vi "Get Local Chassis Slots Configuration.vi"(8 "error in (no error)":errorcluster, 11 "Item Ref in":T2 format="%.0x") -> (0 "error out":errorcluster, 2 "Slots Configuration":T1[](array[typedef]), 3 "Item Ref out":T2 format="%.0x")   [LabVIEW 2027, in "SEECD System Explorer.lvlib"]
doc: "This VI lists the module(s) configured in Local Chassis. GUIDs are used to create the list. The output is a list of Slot Number."
uses:
  SEECD System Explorer.lvlib
  <vilib>/NI VeriStand/Custom Device API/Custom Device Item Ref.ctl
  Type Defs/Slot Programming Mode.ctl
  Shared/Globals/Scan Engine GUIDs.vi
  <vilib>/NI VeriStand/Custom Device Tools/Custom Device Utility Library/NI VeriStand - Search for Item by GUID.vi
  Shared/Globals/Property Strings.vi
  <vilib>/NI VeriStand/Custom Device Tools/Custom Device Utility Library/Custom Device Utility Library.lvlib
  Shared/SEECD Shared.lvlib
  <vilib>/NI VeriStand/Custom Device API/Custom Device API.lvlib
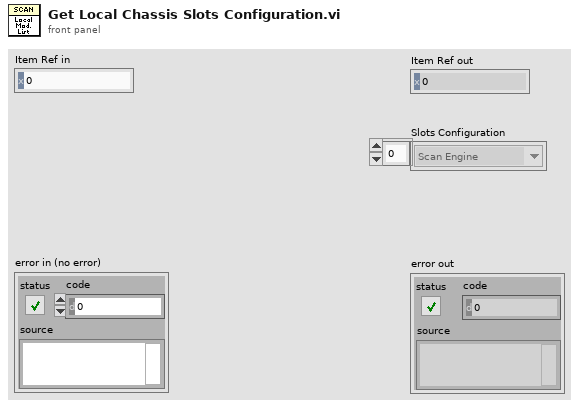
[diagram p1: front panel]
types:
  T1 = typedef "SEECD System Explorer.lvlib/Slot Programming Mode.ctl" = enum16{"Don't Modify", "Scan Engine", "LabVIEW FPGA", "NI-DAQmx"}
  T2 = typedef "Custom Device API.lvlib/Custom Device Item Ref.ctl" = u64
  T3 = typedef "Custom Device API.lvlib/Custom Device Item Info.ctl" = cluster{"Name":string, "Is Channel":bool, "GUID":string, "Is Waveform":bool}
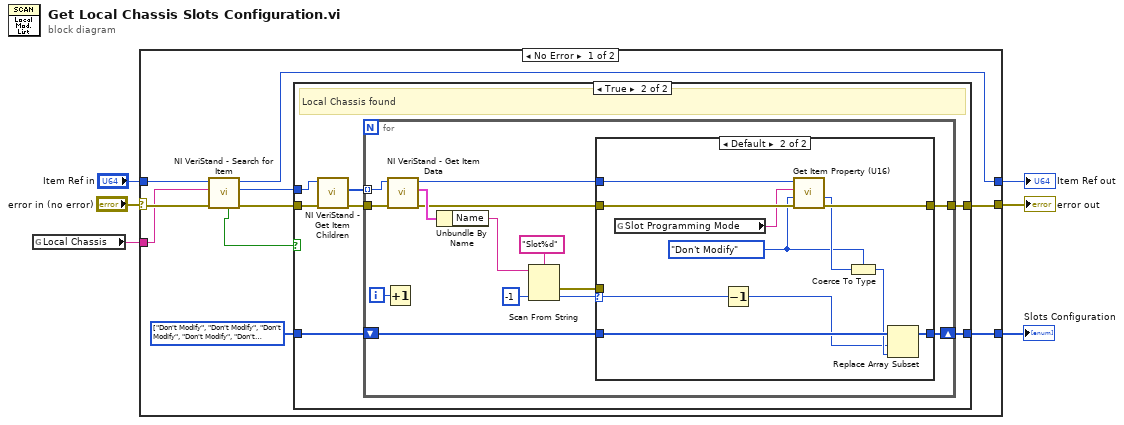
[diagram p0: block diagram]
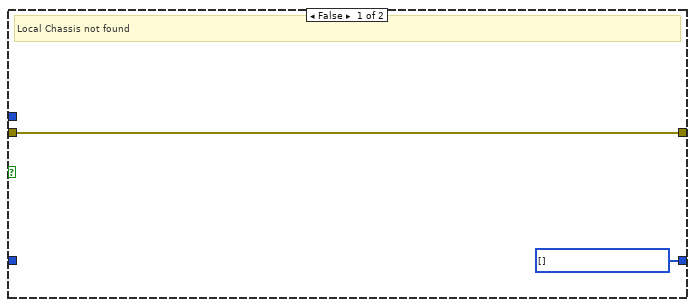
[diagram p2: hidden frame]
diagram:
  n1 = global read "Scan Engine GUIDs.vi" "Local Chassis"() -> (w3:string)
  n2 = case shown="No Error" "error in (no error)" {
    selector: "error in (no error)" -> [w16 w54]
    tunnel: [w9 w54] -> w5
    tunnel: "Item Ref in" -> [w15 w53]
    tunnel: w3 -> [w14 _]
    tunnel: [w10 w53] -> w2
    tunnel: [w8 _] -> w1
    frame No Error {
      w7 = T1[] [enum."Don't Modify", enum."Don't Modify", enum."Don't Modify", enum."Don't Modify", enum."Don't Modify", enum."Don't Modify", enum."Don't Modify", enum."Don't Modify"] items=["Don't Modify", "Scan Engine", "LabVIEW FPGA", "NI-DAQmx"] ("Slots Configuration")
      n3 = call-poly <vilib>:"NI VeriStand - Search for Item.vi"("error in"=w16, "Item GUID"=w14, "Section Ref in"=w15) -> ("error out"=w12:errorcluster, "Item Ref"=w11:T2, "Section Ref out"=w10:T2, "Found"=w13:bool)  [unwired: 5 in]
      n4 = case shown="True" w13 {
        tunnel: w12 -> [w18 w24]
        tunnel: w11 -> [_ w23]
        tunnel: [w18 w25] -> w9
        tunnel: [w17 w19] -> w8
        tunnel: w7 -> [_ w20]
        frame False {
          w17 = T1[] [] items=["Don't Modify", "Scan Engine", "LabVIEW FPGA", "NI-DAQmx"] ("Slots Configuration")
          # "Local Chassis not found"
        }
        frame True {
          # "Local Chassis found"
          n5 = call <vilib>:"NI VeriStand - Get Item Children.vi"("error in (no error)"=w24, "Item Ref in"=w23) -> ("error out"=w21:errorcluster, "Child Refs"=w22:T2[])  [unwired: 6 in, 2 out]
          n6 = for {
            tunnel: [w39] -> w25
            tunnel: w22 -> [w37] mode=indexing
            tunnel: w21 -> [w38]
            shift-right: [w31] -> w19
            shift-left: w20 -> [w32]
            i -> [w33]
            n7 = Increment(x=w33) -> ()  [unwired: 1 out]
            n8 = call <vilib>:"NI VeriStand - Get Item Data.vi"("error in (no error)"=w38, "Item Ref in"=w37) -> ("error out"=w35:errorcluster, "Item Info"=w36:T3, "Item Ref out"=w34:T2)  [unwired: 6 in, 1 out]
            n9 = Unbundle By Name(w36) -> ("Name"=w30:string)
            n10 = Scan From String(format string="Slot%d", input string=w30, default 1=-1 ("default value 1")) -> (error out=w26:errorcluster, output 1=w28:i32)  [unwired: 2 in, 2 out]
            n11 = case shown="Default" w28 {
              selector: w28 -> [_ w42]
              tunnel: w35 -> [w41 w52]
              tunnel: [w41 w51] -> w39
              tunnel: [w40 w45] -> w31
              tunnel: w34 -> [_ w47]
              tunnel: w32 -> [w40 w46]
              tunnel: w26 -> [_ _]
              frame -1 {
              }
              frame Default {
                w49 = Slot_Programming_Mode."Don't Modify" ("Slot Programming Mode 2")
                n12 = global read "Property Strings.vi" "Slot Programming Mode"() -> (w48:string)
                n13 = Decrement(x=w42) -> (x-1=w43:i32)
                n14 = call <vilib>:"Get Item Property (U16).vi"("error in (no error)"=w52, "Default Value"=w49, "Property Name"=w48, "Item Ref in"=w47) -> ("error out"=w51:errorcluster, "Value"=w50:u16)  [unwired: 4 in, 2 out]
                n15 = Coerce To Type(0:w50, 1:w49) -> (2:w44:T1)
                n16 = Replace Array Subset(array=w46, new element=w44, index=w43) -> (w45:T1[])
              }
            }
          }
        }
      }
    }
    frame Error {
    }
  }
  "Item Ref out" <- w2
  "error out" <- w5
  "Slots Configuration" <- w1
